vi "Func - Get list of arguments.vi"(7 "InstanceRef":T1, 8 "error in":bool, 9 "max arg num":i32=100, 10 "min arg num":i32=1, 11 "arg list":T2[](array[typedef])) -> (0 "error out":bool, 1 "type list":u32[](array[numeric]), 2 "str list":string[](array[string]), 3 "num list":dbl[](array[numeric]) format="%.3f")   [LabVIEW 2021]
doc: "This VI returns the values of function arguments. It verifies the number of actual arguments but does not check argument data types. Refer to the VI help for more details.\n\n<b>arg list</b> specifies the list of function arguments passed to a FuncVI. Wire it to the same terminal on the FuncVI block diagram.\n\n<b>min arg num</b> and <b>max arg num</b> specify the minimum and the maximum number of arguments allowed.\n\nFor more information, see help for this VI.\n\n::: CalcExpress Toolkit :::\nCopyright (c) 2000-2026 Konstantin Shifershteyn. All rights reserved."
uses:
  cetypes.llb/CalcExpress Function Argument Info.ctl
  cetypes.llb/CalcExpress Instance RefNum.ctl
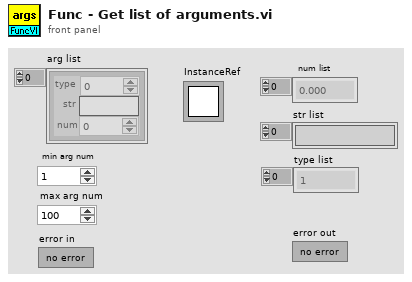
[diagram p1: front panel]
types:
  T1 = typedef "CalcExpress Instance RefNum.ctl" = refnum<k1>
  T2 = typedef "CalcExpress Function Argument Info.ctl" = cluster{"type":u32, "str":string, "num":dbl}
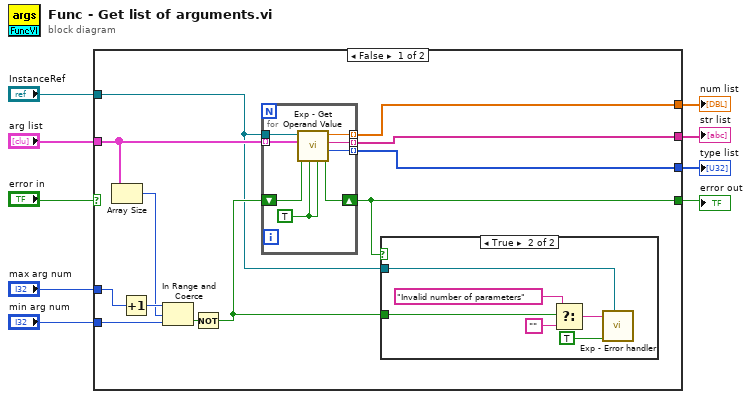
[diagram p0: block diagram]
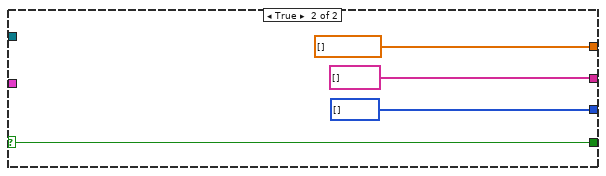
[diagram p3: hidden frame]
diagram:
  n1 = case shown="False" "error in" {
    selector: "error in" -> [_ w36]
    tunnel: [w17 w36] -> w9
    tunnel: [w16 u32[] [] ("type list")] -> w8
    tunnel: [w15 string[] [] ("str list")] -> w7
    tunnel: [w14 dbl[] [] ("num list")] -> w6
    tunnel: "min arg num" -> [w13 _]
    tunnel: "max arg num" -> [w12 _]
    tunnel: "InstanceRef" -> [w10 _]
    tunnel: "arg list" -> [w11 _]
    frame False {
      n2 = Array Size(array=w11) -> (size(s)=w19:i32)
      n3 = Increment(x=w12) -> (x+1=w20:i32)
      n4 = In Range and Coerce(upper limit=w20, x=w19, lower limit=w13) -> (In Range?=w18:bool)  [unwired: 1 out]
      n5 = Not(x=w18) -> (.not. x?=w21:bool)
      n6 = for {
        tunnel: w11 -> [w26] mode=indexing
        shift-right: [w28] -> w17
        shift-left: w21 -> [w29]
        tunnel: [w27] -> w14 mode=indexing
        tunnel: w10 -> [w25]
        tunnel: [w24] -> w15 mode=indexing
        tunnel: [w23] -> w16 mode=indexing
        w22 = TRUE ("may be string ? (F)")
        n7 = call "Exp - Get Operand Value.vi"("ena complex? (F)"=w22, "ena string? (F)"=w22, "error in"=w29, "op info"=w26, "InstanceRef"=w25) -> ("error out"=w28:bool, "type"=w23:u32, "str"=w24:string, "num"=w27:dbl)  [unwired: 1 in]
      }
      n8 = case shown="True" w17 {
        tunnel: w21 -> [_ w35]
        tunnel: w10 -> [_ w30]
        frame False {
        }
        frame True {
          n9 = Select(t="Invalid number of parameters" ("ErrStr"), s=w35, f="") -> (s? t:f=w31:string)
          n10 = call "Exp - Error handler.vi"("InstanceRef"=w30, "error in"=TRUE, "error message in"=w31) -> ()  [unwired: 6 in, 3 out]
        }
      }
    }
    frame True {
    }
  }
  "error out" <- w9
  "num list" <- w6
  "str list" <- w7
  "type list" <- w8
